vi "simulate-dashboard.vi"() -> ()   [LabVIEW 2019]
uses:
  <vilib>/Rock Robotics/WPI/ThirdParty/JAS_Junk/TrajLib/TypeDef/CHASSIS_SPEEDS.ctl
  <vilib>/Rock Robotics/WPI/ThirdParty/JAS_Junk/TrajLib/TypeDef/POSE2D.ctl
  <vilib>/Rock Robotics/WPI/ThirdParty/JAS_Junk/TrajLib/TypeDef/TRANSLATION2D.ctl
  <vilib>/Rock Robotics/WPI/ThirdParty/JAS_Junk/TrajLib/TypeDef/ROTATION2D.ctl
  <vilib>/Rock Robotics/WPI/ThirdParty/JAS_Junk/TrajLib/TypeDef/TRAJ_STATE.ctl
  <vilib>/Rock Robotics/WPI/ThirdParty/JAS_Junk/TrajLib/TypeDef/TRAJECTORY.ctl
  Swerve_Drive_System/SDO_DRIVE_GLOBALS.vi
  Simulation/SDO_SIM_SIM_Globals.vi
  Trajectory Following/SDO_TRAJECTORY_GLOBALS.vi
  Vision_Interface/SDO_Vision_Globals.vi
  <vilib>/Rock Robotics/WPI/ThirdParty/JAS_Junk/TrajLib/Trajectory_Library.lvlib
panel:
  in  "Tab Control":T1(tab)
  out "Mod Swerve in Deadband 2":bool
  out "Battery Voltage":dbl(graph)
  out "Swerve Motor Demands":T2(graph)
  out "Drive Motor Demands":T2(graph)
  out "Swerve Module Devices":T3(array[cluster])
  out "GyroReading_Degreees":dbl format="%15.3f"
  out "Encoder Distances":dbl[](array[numeric]) format="%17.2f"
  out "Encoder Velocities":dbl[](array[numeric]) format="%17.2f"
  out "Motor Demands":dbl[](array[numeric]) format="%17.2f"
  out "Battery Volts":dbl format="%16.2f"
  out "Mod Wheel \nSpeed Dmd":dbl[](array[numeric]) format="%17.3f"
  out "Swerve Drive Motor output":T4(graph)
  out "Swerve Drive Speed M/S":T5(graph)
  out "Swerve Drive Speed Error  M/S":T6(graph)
  out "Closed Loop Control":bool
  out "Orientation Angle Dmd_Rad":dbl format="%17.3f"
  out "Drv Chassis Adj Velocity DmD":T7 {"vOmega" format="%10.3f"; "vY" format="%10.3f"; "vX" format="%10.3f"}
  out "GyroHeading_Radians":dbl format="%17.2f"
  out "Orientation Angle Error_Rad":dbl format="%17.3f"
  out "Orientation Correct CO":dbl format="%17.3f"
  out "Swerve Chassis Speed":T7 {"vOmega" format="%10.3f"; "vY" format="%10.3f"; "vX" format="%10.3f"}
  out "Mod Swerve in Deadband":bool
  out "Mod Wheel Out":dbl[](array[numeric]) format="%17.3f"
  out "Mod Wheel \nSpeed M/S":dbl[](array[numeric]) format="%17.3f"
  out "Mod Wheel Speed Err":dbl[](array[numeric]) format="%17.3f"
  out "Opt Mod Wheel \nSpeed Dmd":dbl[](array[numeric]) format="%17.3f"
  out "Swerve Pos Dmd\nRadians":dbl[](array[numeric]) format="%17.3f"
  out "Optimized Swerve\nPos Dmd":dbl[](array[numeric]) format="%17.3f"
  out "Sweve Module Motor Output":T8(graph)
  out "Swerve Modue Position Radians":T5(graph)
  out "Swerve Module Position Error\nRadians":T9(graph)
  out "Closed Loop Control 2":bool
  out "Mod Swerve in Deadband 3":bool
  out "Mod Swerve Err  Radians":dbl[](array[numeric]) format="%17.3f"
  out "Mod Swerve Motor Out":dbl[](array[numeric]) format="%17.3f"
  out "Mod Pos Radians":dbl[](array[numeric]) format="%17.3f"
  out "Mod Swerve On Targ":bool[](array[boolean])
  out "Vision Pose":T10={"TRANSLATION"={"X"=0.0, "Y"=0.0}, "ROTATION"={"VALUE"=0.0, "COS"=1.0, "SIN"=0.0}} {"ROTATION"."SIN" format="%13.4f"; "ROTATION"."COS" format="%13.4f"; "ROTATION"."VALUE" format="%13.4f"; "TRANSLATION"."Y" format="%14.3f"; "TRANSLATION"."X" format="%14.3f"}
  out "Vision\nPose":bool
  out "Trajectory Status":T13(graph)
  out "Trajectory Execution \nClosed Loop":bool
  out "Mod Swerve in \nDeadband 3":bool
  out "Trajectory Error":T14(graph)
  out "Traj_OnTarget":bool
  out "Traj Heading Dmd Deg":dbl format="%17.2f"
  out "Traj Final Heading Dmd Deg":dbl format="%17.2f"
  out "Traj Sample Time Sec":dbl format="%17.2f"
  out "Traj Rot Vel FF Rad/Sec":dbl format="%17.2f"
  out "Relative Trajectory Pose":T10={"TRANSLATION"={"X"=0.0, "Y"=0.0}, "ROTATION"={"VALUE"=0.0, "COS"=1.0, "SIN"=0.0}} {"ROTATION"."SIN" format="%13.4f"; "ROTATION"."COS" format="%13.4f"; "ROTATION"."VALUE" format="%13.4f"; "TRANSLATION"."Y" format="%14.3f"; "TRANSLATION"."X" format="%14.3f"}
  out "Absolute Odometry \nPose":T10={"TRANSLATION"={"X"=0.0, "Y"=0.0}, "ROTATION"={"VALUE"=0.0, "COS"=1.0, "SIN"=0.0}} {"ROTATION"."SIN" format="%13.4f"; "ROTATION"."COS" format="%13.4f"; "ROTATION"."VALUE" format="%13.4f"; "TRANSLATION"."Y" format="%14.3f"; "TRANSLATION"."X" format="%14.3f"}
  out "Current Trajectory State":T15={"TimeSeconds"=0.0, "Velocity"=0.0, "Acceleration"=0.0, "POSE"={"TRANSLATION"={"X"=0.0, "Y"=0.0}, "ROTATION"={"VALUE"=0.0, "COS"=1.0, "SIN"=0.0}}, "Curvature"=0.0} {"POSE"."ROTATION"."SIN" format="%13.4f"; "POSE"."ROTATION"."COS" format="%13.4f"; "POSE"."ROTATION"."VALUE" format="%13.4f"; "POSE"."TRANSLATION"."Y" format="%14.3f"; "POSE"."TRANSLATION"."X" format="%14.3f"}
  out "Other ABS Odometry\nPose":T10={"TRANSLATION"={"X"=0.0, "Y"=0.0}, "ROTATION"={"VALUE"=0.0, "COS"=1.0, "SIN"=0.0}} {"ROTATION"."SIN" format="%13.4f"; "ROTATION"."COS" format="%13.4f"; "ROTATION"."VALUE" format="%13.4f"; "TRANSLATION"."Y" format="%14.3f"; "TRANSLATION"."X" format="%14.3f"}
  out "Absolue Trajectory":cluster{dbl[], dbl[]}(graph)
  out "Absolute Trajectory":T16 {"States"."POSE"."ROTATION"."SIN" format="%13.4f"; "States"."POSE"."ROTATION"."COS" format="%13.4f"; "States"."POSE"."ROTATION"."VALUE" format="%13.4f"; "States"."POSE"."TRANSLATION"."Y" format="%14.3f"; "States"."POSE"."TRANSLATION"."X" format="%14.3f"; "TotalTImeSecs" format="%20.3f"}
  out "Relative Trajectory":cluster{dbl[], dbl[]}(graph)
  # "SIMULATION"
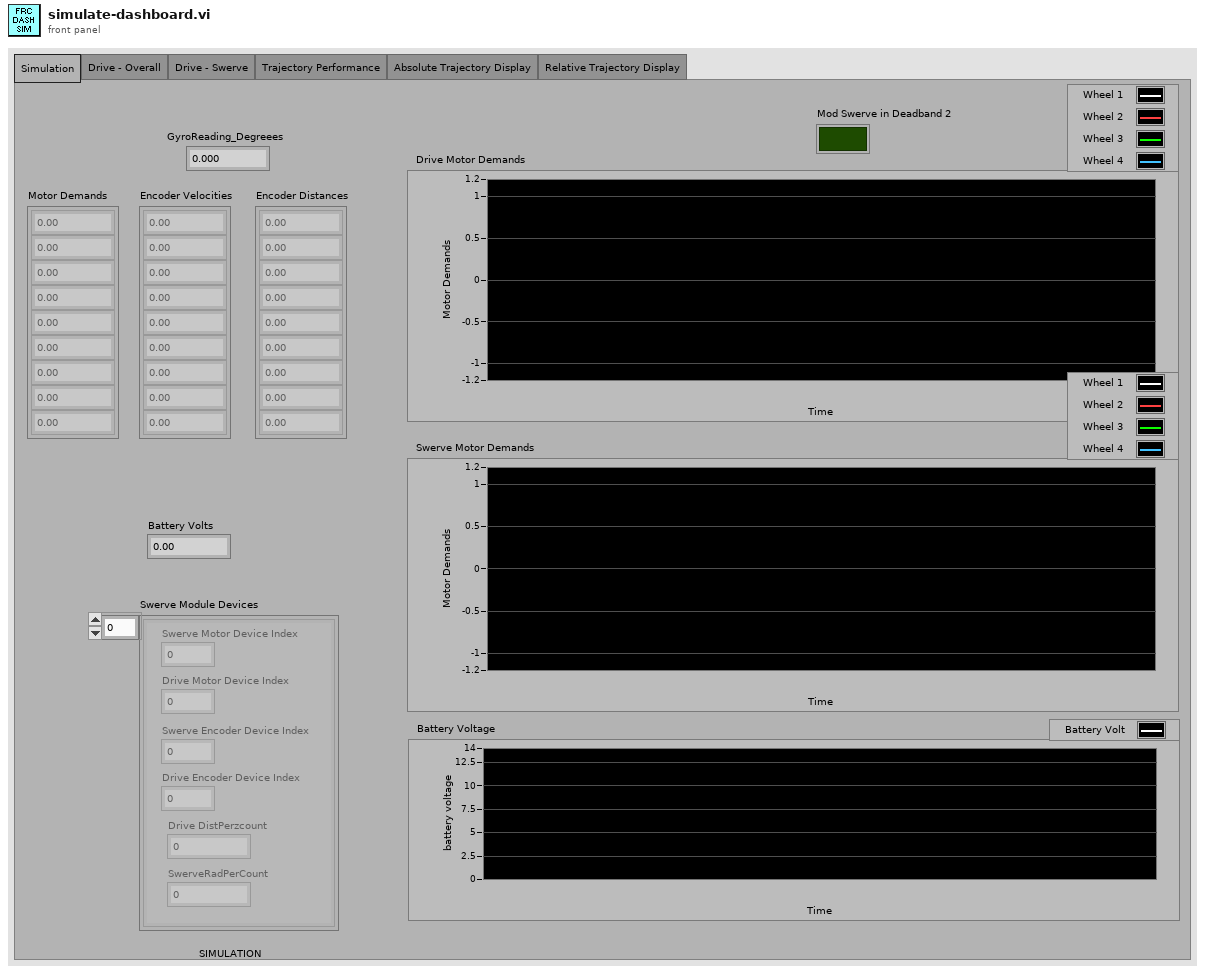
[diagram p1: front panel]
types:
  T1 = enum32{"Simulation", "Drive - Overall", "Drive - Swerve", "Trajectory Performance", "Absolute Trajectory Display", "Relative Trajectory Display"}
  T2 = cluster{"Motor Dmd":dbl, "Motor Dmd":dbl, "Motor Dmd":dbl, "Motor Dmd":dbl}
  T3 = cluster{"Swerve Motor Device Index":i32, "Drive Motor Device Index":i32, "Swerve Encoder Device Index":i32, "Drive Encoder Device Index":i32, "Drive DistPerzcount":dbl, "SwerveRadPerCount":dbl}[]
  T4 = cluster{"Mod Wheel Out[0]":dbl, "Mod Wheel Out[1]":dbl, "Mod Wheel Out[2]":dbl, "Mod Wheel Out[3]":dbl}
  T5 = cluster{"Angle RADIANS":dbl, "Angle RADIANS":dbl, "Angle RADIANS":dbl, "Distance M":dbl}
  T6 = cluster{"Mod Wheel Speed Err[0]":dbl, "Mod Wheel Speed Err[1]":dbl, "Mod Wheel Speed Err[2]":dbl, "Mod Wheel Speed Err[3]":dbl}
  T7 = typedef "Trajectory_Library.lvlib/CHASSIS_SPEEDS.ctl" = cluster{"vX":dbl, "vY":dbl, "vOmega":dbl}
  T8 = cluster{"Mod Swerve Out[0]":dbl, "Mod Swerve Out[1]":dbl, "Mod Swerve Out[2]":dbl, "Mod Swerve Out[3]":dbl}
  T9 = cluster{"Mod Swerve Err[0]":dbl, "Mod Swerve Err[1]":dbl, "Mod Swerve Err[2]":dbl, "Mod Swerve Err[3]":dbl}
  T10 = typedef "Trajectory_Library.lvlib/POSE2D.ctl" = cluster{"TRANSLATION":T11, "ROTATION":T12}
  T11 = typedef "Trajectory_Library.lvlib/TRANSLATION2D.ctl" = cluster{"X":dbl, "Y":dbl}
  T12 = typedef "Trajectory_Library.lvlib/ROTATION2D.ctl" = cluster{"VALUE":dbl, "COS":dbl, "SIN":dbl}
  T13 = cluster{dbl, dbl, dbl, "Traj_Sample_Time_Sec":dbl}
  T14 = cluster{"Traj X Err":dbl, "Traj Y Err":dbl, "Traj Heading Err":dbl}
  T15 = typedef "Trajectory_Library.lvlib/TRAJ_STATE.ctl" = cluster{"TimeSeconds":dbl, "Velocity":dbl, "Acceleration":dbl, "POSE":T10, "Curvature":dbl}
  T16 = typedef "Trajectory_Library.lvlib/TRAJECTORY.ctl" = cluster{"TotalTImeSecs":dbl, "States":T15[]}
  T17 = cluster{"Traj X Err_FT":dbl, "Traj Y Err_FT":dbl, "Traj Heading Err_DEG":dbl}
  T18 = typedef "Trajectory_Library.lvlib/SWERVE_DRIVE_MODULE_POSITION.ctl" = cluster{"Distance":dbl, "Angle":T12, "P":bool}
  T19 = typedef "Trajectory_Library.lvlib/SWERVE_DRIVE_MODULE_STATE.ctl" = cluster{"Speed":dbl, "Angle":T12}
  T20 = cluster{"Angle RADIANS":dbl, "Angle RADIANS":dbl, "Angle RADIANS":dbl, "Angle RADIANS":dbl}
  T21 = cluster{"Speed M/S":dbl, "Speed M/S":dbl, "Speed M/S":dbl, "Speed M/S":dbl}
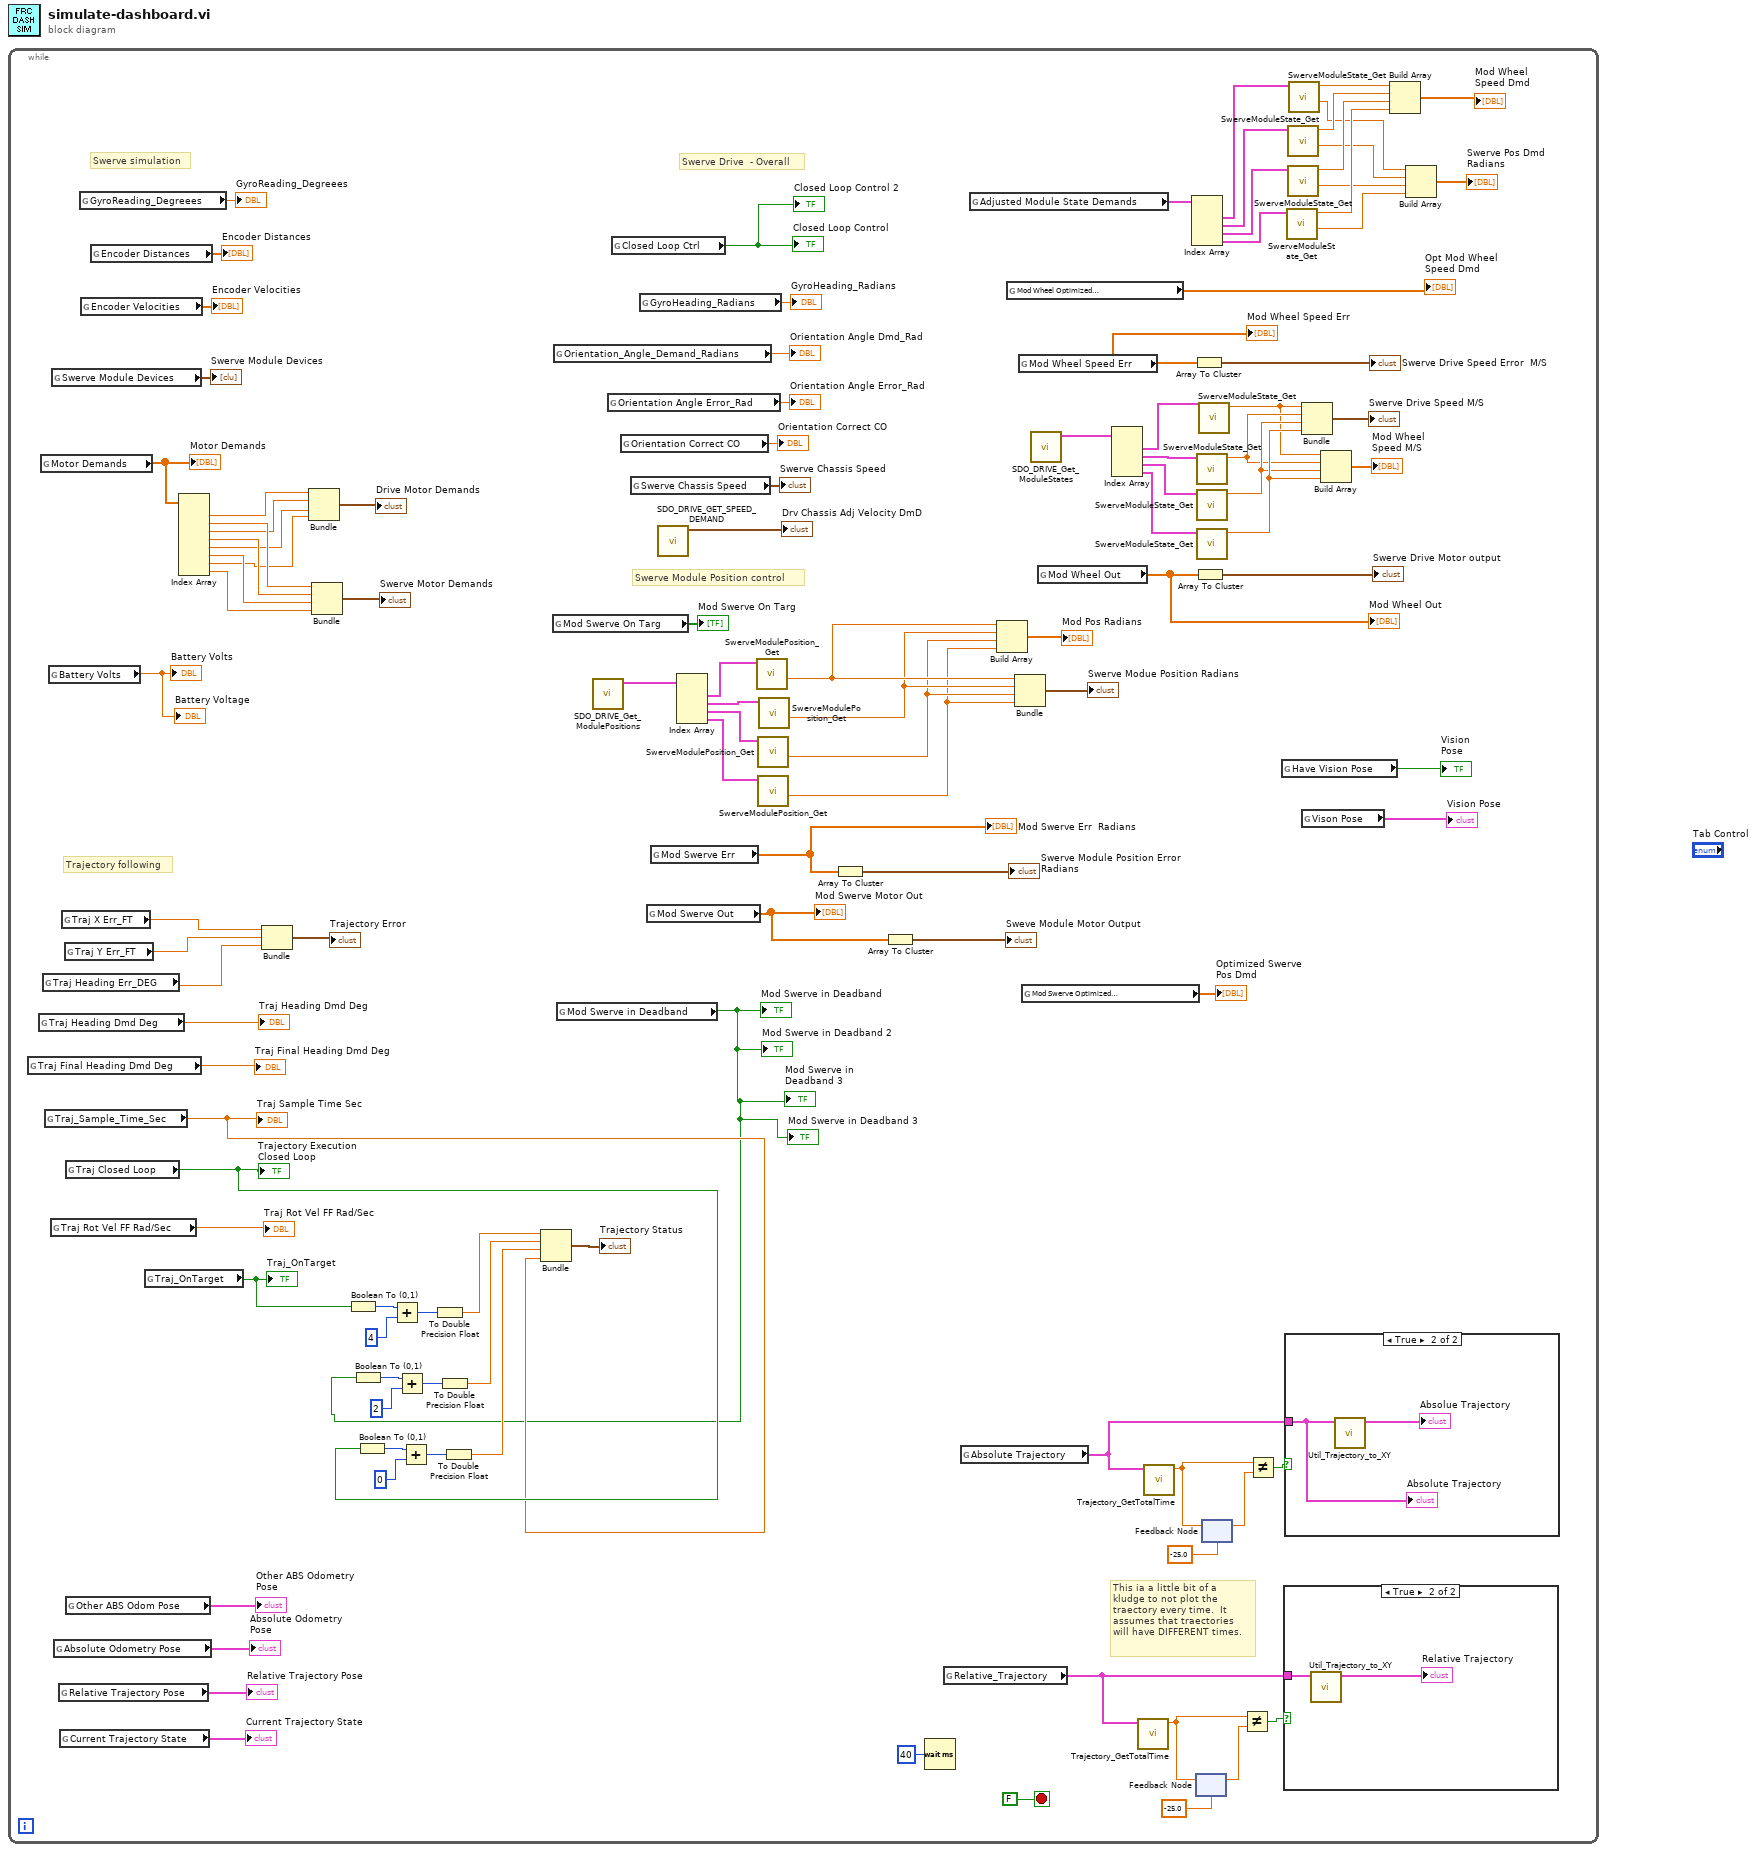
[diagram p0: block diagram]
diagram:
  n1 = while {
    stop <- FALSE stop-if-true
    # "Swerve Module Position control"
    # "This ia a little bit of a \nkludge to not plot the\ntraectory every time.  It \nassumes that traectories\nwill have DIFFERENT times."
    # "Trajectory following"
    # "Swerve simulation"
    # "Swerve Drive  - Overall"
    n2 = global read "SDO_TRAJECTORY_GLOBALS.vi" "Traj Final Heading Dmd Deg"() -> (→"Traj Final Heading Dmd Deg":dbl)
    n3 = global read "SDO_TRAJECTORY_GLOBALS.vi" "Traj Heading Dmd Deg"() -> (→"Traj Heading Dmd Deg":dbl)
    n4 = global read "SDO_SIM_SIM_Globals.vi" "Motor Demands"() -> (w100:dbl[])
    "Motor Demands" <- w100
    n5 = global read "SDO_TRAJECTORY_GLOBALS.vi" "Traj Heading Err_DEG"() -> (w87:dbl)
    n6 = global read "SDO_TRAJECTORY_GLOBALS.vi" "Traj_Sample_Time_Sec"() -> (w68:dbl)
    "Traj Sample Time Sec" <- w68
    n7 = global read "SDO_SIM_SIM_Globals.vi" "Battery Volts"() -> (→"Battery Volts" →"Battery Voltage":dbl)
    n8 = global read "SDO_TRAJECTORY_GLOBALS.vi" "Traj Rot Vel FF Rad/Sec"() -> (→"Traj Rot Vel FF Rad/Sec":dbl)
    n9 = global read "SDO_SIM_SIM_Globals.vi" "Swerve Module Devices"() -> (→"Swerve Module Devices":T3)
    n10 = global read "SDO_TRAJECTORY_GLOBALS.vi" "Absolute Odometry Pose"() -> (→"Absolute Odometry \nPose":T10)
    n11 = global read "SDO_TRAJECTORY_GLOBALS.vi" "Relative Trajectory Pose"() -> (→"Relative Trajectory Pose":T10)
    n12 = global read "SDO_TRAJECTORY_GLOBALS.vi" "Current Trajectory State"() -> (→"Current Trajectory State":T15)
    n13 = global read "SDO_TRAJECTORY_GLOBALS.vi" "Traj X Err_FT"() -> (w89:dbl)
    n14 = global read "SDO_TRAJECTORY_GLOBALS.vi" "Traj Y Err_FT"() -> (w88:dbl)
    n15 = global read "SDO_TRAJECTORY_GLOBALS.vi" "Traj Closed Loop"() -> (w70:bool)
    "Trajectory Execution \nClosed Loop" <- w70
    n16 = global read "SDO_TRAJECTORY_GLOBALS.vi" "Other ABS Odom Pose"() -> (→"Other ABS Odometry\nPose":T10)
    n17 = global read "SDO_SIM_SIM_Globals.vi" "GyroReading_Degreees"() -> (→"GyroReading_Degreees":dbl)
    n18 = global read "SDO_SIM_SIM_Globals.vi" "Encoder Velocities"() -> (→"Encoder Velocities":dbl[])
    n19 = global read "SDO_SIM_SIM_Globals.vi" "Encoder Distances"() -> (→"Encoder Distances":dbl[])
    n20 = global read "SDO_TRAJECTORY_GLOBALS.vi" "Traj_OnTarget"() -> (w82:bool)
    "Traj_OnTarget" <- w82
    n21 = Index Array(array=w100) -> (element #1=w99:dbl, element #2=w98:dbl, element #3=w97:dbl, element #4=w96:dbl, element #5=w95:dbl, element #6=w94:dbl, element #7=w93:dbl, element #8=w92:dbl)  [unwired: 8 in]
    n22 = Bundle("Traj X Err_FT"=w89, "Traj Y Err_FT"=w88, "Traj Heading Err_DEG"=w87) -> (→"Trajectory Error":T17)  [unwired: 1 in]
    n23 = Bundle("Motor Dmd"=w99, "Motor Dmd"=w97, "Motor Dmd"=w95, "Motor Dmd"=w93) -> (→"Drive Motor Demands":T2)  [unwired: 1 in]
    n24 = Bundle("Motor Dmd"=w98, "Motor Dmd"=w96, "Motor Dmd"=w94, "Motor Dmd"=w92) -> (→"Swerve Motor Demands":T2)  [unwired: 1 in]
    n25 = Boolean To (0,1)(Boolean=w82) -> (0, 1=w80:i16)
    n26 = Boolean To (0,1)(Boolean=w70) -> (0, 1=w73:i16)
    n27 = Add(x=w80, y=i16 4) -> (x+y=w79:i16)
    n28 = Add(x=w73, y=i16 0) -> (x+y=w72:i16)
    n29 = To Double Precision Float(number=w79) -> (double precision float=w81:dbl)
    n30 = To Double Precision Float(number=w72) -> (double precision float=w69:dbl)
    n31 = global read "SDO_DRIVE_GLOBALS.vi" "Mod Swerve On Targ"() -> (→"Mod Swerve On Targ":bool[])
    n32 = global read "SDO_DRIVE_GLOBALS.vi" "Orientation_Angle_Demand_Radians"() -> (→"Orientation Angle Dmd_Rad":dbl)
    n33 = global read "SDO_DRIVE_GLOBALS.vi" "Mod Swerve in Deadband"() -> (w43:bool)
    "Mod Swerve in Deadband" <- w43
    "Mod Swerve in Deadband 2" <- w43
    "Mod Swerve in \nDeadband 3" <- w43
    "Mod Swerve in Deadband 3" <- w43
    n34 = Boolean To (0,1)(Boolean=w43) -> (0, 1=w77:i16)
    n35 = Add(x=w77, y=i16 2) -> (x+y=w76:i16)
    n36 = To Double Precision Float(number=w76) -> (double precision float=w74:dbl)
    n37 = Bundle(w81, w74, w69, "Traj_Sample_Time_Sec"=w68) -> (→"Trajectory Status":T13)  [unwired: 1 in]
    n38 = call "SDO_DRIVE_Get_ModulePositions.vi"() -> ("Swerve Module Positions"=w62:T18[])  [unwired: 11 in]
    n39 = global read "SDO_DRIVE_GLOBALS.vi" "Orientation Angle Error_Rad"() -> (→"Orientation Angle Error_Rad":dbl)
    n40 = global read "SDO_DRIVE_GLOBALS.vi" "Closed Loop Ctrl"() -> (→"Closed Loop Control" →"Closed Loop Control 2":bool)
    n41 = global read "SDO_DRIVE_GLOBALS.vi" "Orientation Correct CO"() -> (→"Orientation Correct CO":dbl)
    n42 = global read "SDO_DRIVE_GLOBALS.vi" "Swerve Chassis Speed"() -> (→"Swerve Chassis Speed":T7)
    n43 = global read "SDO_DRIVE_GLOBALS.vi" "GyroHeading_Radians"() -> (→"GyroHeading_Radians":dbl)
    n44 = global read "SDO_DRIVE_GLOBALS.vi" "Mod Swerve Out"() -> (w31:dbl[])
    "Mod Swerve Motor Out" <- w31
    n45 = global read "SDO_DRIVE_GLOBALS.vi" "Mod Swerve Err"() -> (w57:dbl[])
    "Mod Swerve Err  Radians" <- w57
    n46 = call "SDO_DRIVE_GET_SPEED_DEMAND.vi"() -> ("Drv Chassis Velocity DmD"=→"Drv Chassis Adj Velocity DmD":T7)  [unwired: 11 in]
    n47 = Index Array(array=w62) -> (element #1=w61:T18, element #2=w60:T18, element #3=w59:T18, element #4=w58:T18)  [unwired: 4 in]
    n48 = call <vilib>:"SwerveModulePosition_Get.vi"("Swerve Module Position"=w61) -> ("Angle RADIANS"=w30:dbl)  [unwired: 8 in, 2 out]
    n49 = call <vilib>:"SwerveModulePosition_Get.vi"("Swerve Module Position"=w59) -> ("Angle RADIANS"=w28:dbl)  [unwired: 8 in, 2 out]
    n50 = call <vilib>:"SwerveModulePosition_Get.vi"("Swerve Module Position"=w58) -> ("Angle RADIANS"=w27:dbl)  [unwired: 8 in, 2 out]
    n51 = call <vilib>:"SwerveModulePosition_Get.vi"("Swerve Module Position"=w60) -> ("Angle RADIANS"=w29:dbl)  [unwired: 8 in, 2 out]
    n52 = Array To Cluster(array=w57) -> (cluster=→"Swerve Module Position Error\nRadians":T9)
    n53 = Array To Cluster(array=w31) -> (cluster=→"Sweve Module Motor Output":T8)
    n54 = Wait (ms)(milliseconds to wait=u32 40) -> ()  [unwired: 1 out]
    n55 = global read "SDO_TRAJECTORY_GLOBALS.vi" "Relative_Trajectory"() -> (w45:T16)
    n56 = global read "SDO_TRAJECTORY_GLOBALS.vi" "Absolute Trajectory"() -> (w51:T16)
    n57 = global read "SDO_DRIVE_GLOBALS.vi" "Adjusted Module State Demands"() -> (w20:T19[])
    n58 = Build Array(w30, w29, w28, w27) -> (→"Mod Pos Radians":dbl[])
    n59 = global read "SDO_DRIVE_GLOBALS.vi" "Mod Wheel Optimized \nDmd"() -> (→"Opt Mod Wheel \nSpeed Dmd":dbl[])
    n60 = Bundle("Angle RADIANS"=w30, "Angle RADIANS"=w29, "Angle RADIANS"=w28, "Angle RADIANS"=w27) -> (→"Swerve Modue Position Radians":T20)  [unwired: 1 in]
    n61 = global read "SDO_DRIVE_GLOBALS.vi" "Mod Wheel Speed Err"() -> (w56:dbl[])
    "Mod Wheel Speed Err" <- w56
    n62 = global read "SDO_DRIVE_GLOBALS.vi" "Mod Swerve Optimized\nDmd"() -> (→"Optimized Swerve\nPos Dmd":dbl[])
    n63 = call "SDO_DRIVE_Get_ModuleStates.vi"() -> ("Swerve Module States"=w40:T19[])  [unwired: 11 in]
    n64 = global read "SDO_DRIVE_GLOBALS.vi" "Mod Wheel Out"() -> (w34:dbl[])
    "Mod Wheel Out" <- w34
    n65 = Index Array(array=w40) -> (element #1=w38:T19, element #2=w39:T19, element #3=w37:T19, element #4=w36:T19)  [unwired: 4 in]
    n66 = call <vilib>:"Trajectory_GetTotalTime.vi"("TRAJECTORY"=w45) -> ("TotalTime_Sec"=w48:dbl)  [unwired: 10 in]
    n67 = call <vilib>:"Trajectory_GetTotalTime.vi"("TRAJECTORY"=w51) -> ("TotalTime_Sec"=w53:dbl)  [unwired: 10 in]
    n68 = Index Array(array=w20) -> (element #1=w19:T19, element #2=w18:T19, element #3=w17:T19, element #4=w16:T19)  [unwired: 4 in]
    n69 = Array To Cluster(array=w56) -> (cluster=→"Swerve Drive Speed Error  M/S":T6)
    n70 = Array To Cluster(array=w34) -> (cluster=→"Swerve Drive Motor output":T4)
    n71 = feedback #1(-25.0 ("TotalTime_Sec")) -> (w47:dbl)
    n72 = feedback-in #1(w48) -> ()
    n73 = call <vilib>:"SwerveModuleState_Get.vi"("Desired State"=w39) -> ("Speed M/S"=w22:dbl)  [unwired: 9 in, 1 out]
    n74 = call <vilib>:"SwerveModuleState_Get.vi"("Desired State"=w37) -> ("Speed M/S"=w23:dbl)  [unwired: 9 in, 1 out]
    n75 = call <vilib>:"SwerveModuleState_Get.vi"("Desired State"=w36) -> ("Speed M/S"=w24:dbl)  [unwired: 9 in, 1 out]
    n76 = call <vilib>:"SwerveModuleState_Get.vi"("Desired State"=w38) -> ("Speed M/S"=w21:dbl)  [unwired: 9 in, 1 out]
    n77 = feedback-in #2(w53) -> ()
    n78 = feedback #2(-25.0 ("TotalTime_Sec")) -> (w52:dbl)
    n79 = Not Equal?(x=w48, y=w47) -> (x != y?=w46:bool)
    n80 = Not Equal?(x=w53, y=w52) -> (x != y?=w50:bool)
    n81 = global read "SDO_Vision_Globals.vi" "Have Vision Pose"() -> (→"Vision\nPose":bool)
    n82 = case shown="True" w46 {
      tunnel: w45 -> [_ w115]
      frame False {
      }
      frame True {
        n83 = call <vilib>:"Util_Trajectory_to_XY.vi"("TRAJECTORY"=w115) -> ("outArrayXY"=→"Relative Trajectory":cluster{dbl[], dbl[]})  [unwired: 10 in]
      }
    }
    n84 = case shown="True" w50 {
      tunnel: w51 -> [_ w117]
      frame False {
      }
      frame True {
        n85 = call <vilib>:"Util_Trajectory_to_XY.vi"("TRAJECTORY"=w117) -> ("outArrayXY"=→"Absolue Trajectory":cluster{dbl[], dbl[]})  [unwired: 10 in]
        "Absolute Trajectory" <- w117
      }
    }
    n86 = call <vilib>:"SwerveModuleState_Get.vi"("Desired State"=w16) -> ("Angle RADIANS"=w6:dbl, "Speed M/S"=w12:dbl)  [unwired: 9 in]
    n87 = call <vilib>:"SwerveModuleState_Get.vi"("Desired State"=w18) -> ("Angle RADIANS"=w8:dbl, "Speed M/S"=w14:dbl)  [unwired: 9 in]
    n88 = call <vilib>:"SwerveModuleState_Get.vi"("Desired State"=w17) -> ("Angle RADIANS"=w7:dbl, "Speed M/S"=w13:dbl)  [unwired: 9 in]
    n89 = call <vilib>:"SwerveModuleState_Get.vi"("Desired State"=w19) -> ("Angle RADIANS"=w9:dbl, "Speed M/S"=w15:dbl)  [unwired: 9 in]
    n90 = Bundle("Speed M/S"=w21, "Speed M/S"=w22, "Speed M/S"=w23, "Speed M/S"=w24) -> (→"Swerve Drive Speed M/S":T21)  [unwired: 1 in]
    n91 = global read "SDO_Vision_Globals.vi" "Vison Pose"() -> (→"Vision Pose":T10)
    n92 = Build Array(w21, w22, w23, w24) -> (→"Mod Wheel \nSpeed M/S":dbl[])
    n93 = Build Array(w15, w14, w13, w12) -> (→"Mod Wheel \nSpeed Dmd":dbl[])
    n94 = Build Array(w9, w8, w7, w6) -> (→"Swerve Pos Dmd\nRadians":dbl[])
  }
